vi "Config Motors NEO.vi"(8 "Reset PIDs":bool, 10 "Operation":T5, 11 "Motors In":T2 {"Steer Scaling" format="%.2f"; "Drive Scaling" format="%.2f"; "Pod Locations (ft)"."Right Back Position" format="%.2f"; "Pod Locations (ft)"."Right Front Position" format="%.2f"; "Pod Locations (ft)"."Left Back Position" format="%.2f"; "Pod Locations (ft)"."Left Front Position" format="%.2f"}) -> (3 "Motors Out":T2 {"Steer Scaling" format="%.2f"; "Drive Scaling" format="%.2f"; "Pod Locations (ft)"."Right Back Position" format="%.2f"; "Pod Locations (ft)"."Right Front Position" format="%.2f"; "Pod Locations (ft)"."Left Back Position" format="%.2f"; "Pod Locations (ft)"."Left Front Position" format="%.2f"})   [LabVIEW 2027]
uses:
  Type Definitions/Hardware/Swerve Drives/(NEO-NEO-ThroughBore-Pigeon2) Swerve.ctl
  <vilib>/REV Custom Controls/REVSparkRefnum.ctl
  Type Definitions/Data/Pod Positions.ctl
  Drive/Implementation/Drive Operations.ctl
  <vilib>/REV Custom Controls/Spark Voltage Compensation.ctl
  38a9160b-f87a-407c-aa95-d3b96145cb37.vi
  c612d860-360b-4606-b7b1-9c6eba82ec37.vi
  <resource>/objmgr/REVSpark.rc
  <vilib>/REVLibDriver/REVLibDriver.lvlib
panel:
  in  "value":bool
  in  "Immediate PID":T1={{"P Gain"=0.0005, "I Gain"=0.0, "D Gain"=0.0, "kV"=0.00175}, "I Zone"=0.0, "Output LImits"={"Min Output"=-1.0, "Max Output"=1.0}}
  in  "Auto Gains":T1={{"P Gain"=0.16, "I Gain"=0.0, "D Gain"=0.0, "kV"=0.78}, "I Zone"=0.0, "Output LImits"={"Min Output"=-1.0, "Max Output"=1.0}}
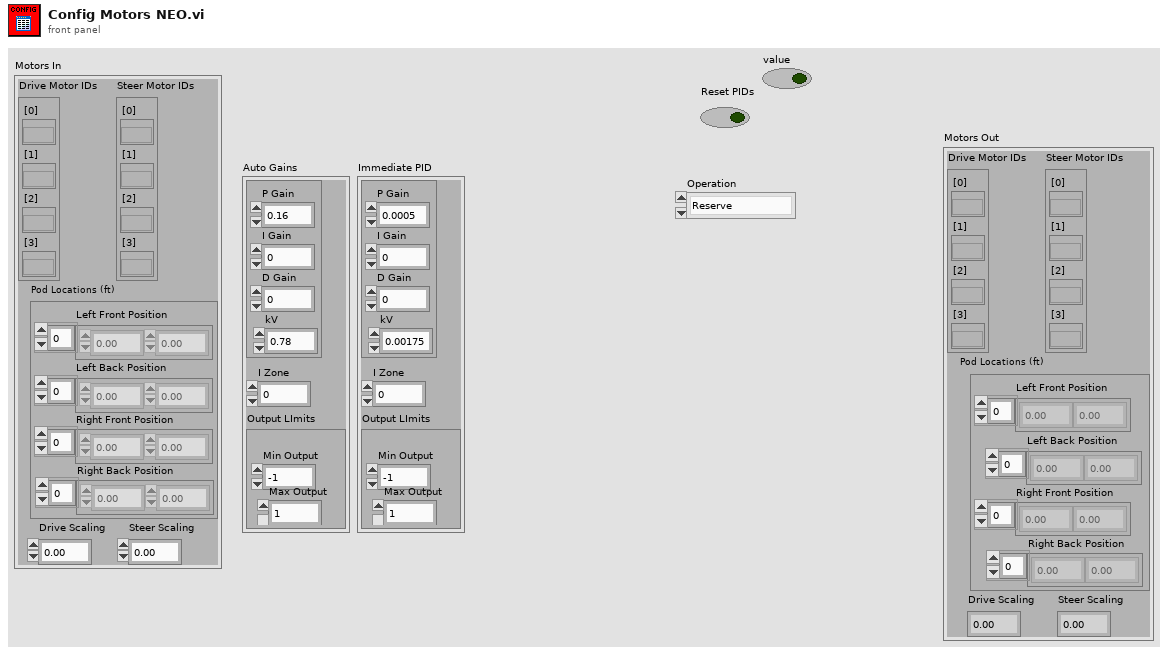
[diagram p1: front panel]
types:
  T1 = cluster{cluster{"P Gain":dbl, "I Gain":dbl, "D Gain":dbl, "kV":dbl}, "I Zone":dbl, "Output LImits":cluster{"Min Output":dbl, "Max Output":dbl}}
  T2 = typedef "(NEO-NEO-ThroughBore-Pigeon2) Swerve.ctl" = cluster{"Drive Motor IDs":cluster{"[0]":T3, "[1]":T3, "[2]":T3, "[3]":T3}, "Steer Motor IDs":cluster{"[0]":T3, "[1]":T3, "[2]":T3, "[3]":T3}, "Pod Locations (ft)":T4, "Drive Scaling":dbl, "Steer Scaling":dbl}
  T3 = typedef "REVLibDriver.lvlib/REVSparkRefnum.ctl" = refnum<k20>
  T4 = typedef "Pod Positions.ctl" = cluster{"Left Front Position":dbl[], "Left Back Position":dbl[], "Right Front Position":dbl[], "Right Back Position":dbl[]}
  T5 = typedef "Drive Operations.ctl" = enum16{"Reserve", "Read Current", "Immediate", "Calibrate", "Auto", "Auto Pickup"}
  T6 = typedef "REVLibDriver.lvlib/Spark Voltage Compensation.ctl" = cluster{"Mode":u32, "Nominal Voltage":dbl}
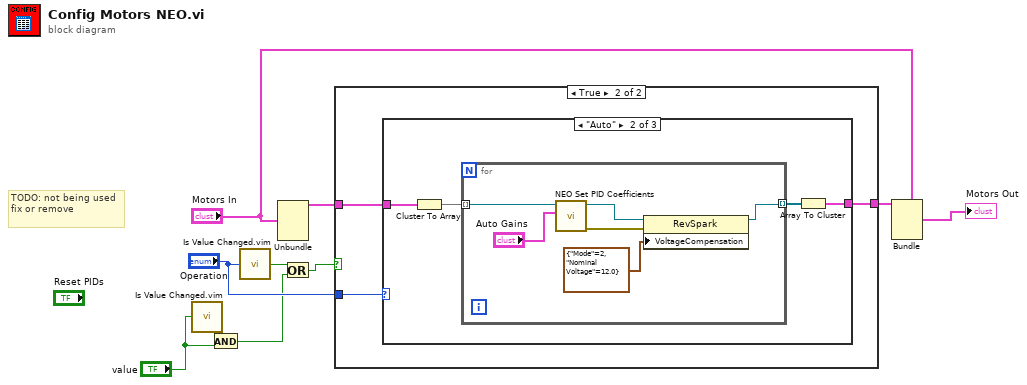
[diagram p0: block diagram]
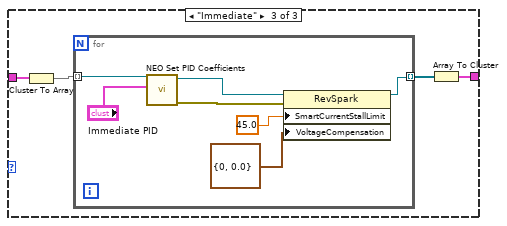
[diagram p4: hidden frame]
diagram:
  # "TODO: not being used\nfix or remove"
  n1 = call "Is Value Changed.vim"("value"="value") -> ("changed or first call?"=w3:bool)
  n2 = And(x=w3, y="value") -> (x .and. y?=w2:bool)
  n3 = call "Is Value Changed.vim"("value"="Operation") -> ("changed or first call?"=w5:bool)
  n4 = Unbundle("Motors In") -> ("Drive Motor IDs"=w10:cluster{"[0]":T3, "[1]":T3, "[2]":T3, "[3]":T3})  [unwired: 4 out]
  n5 = Or(x=w5, y=w2) -> (x .or. y?=w4:bool)
  n6 = case shown="True" w4 {
    tunnel: "Operation" -> [_ w14]
    tunnel: w10 -> [w11 w13]
    tunnel: [w11 w12] -> w8
    frame False {
    }
    frame True {
      n7 = case shown="\"Auto\"" w14 {
        tunnel: w13 -> [w15 w17 w27]
        tunnel: [w15 w18 w28] -> w12
        frame "Reserve", Default {
        }
        frame "Auto" {
          n8 = Cluster To Array(cluster=w17) -> (array=w16:T3[])
          n9 = for {
            tunnel: [w21] -> w19 mode=indexing
            tunnel: w16 -> [w25] mode=indexing
            n10 = call "NEO Set PID Coefficients.vi"("PID Gains"="Auto Gains", "Spark refnum"=w25) -> ("error out"=w20:errorcluster, "Spark refnum out"=w23:T3)  [unwired: 6 in]
            n11 = property class="RevSpark"(reference=w23, error in=w20, "VoltageCompensation"=T6 {"Mode"=2, "Nominal Voltage"=12.0}) -> (reference out=w21:T3)  [unwired: 1 out]
          }
          n12 = Array To Cluster(array=w19) -> (cluster=w18:cluster{"[0]":T3, "[1]":T3, "[2]":T3, "[3]":T3})
        }
        frame "Immediate" {
          n13 = Cluster To Array(cluster=w27) -> (array=w26:T3[])
          n14 = for {
            tunnel: w26 -> [w36] mode=indexing
            tunnel: [w31] -> w29 mode=indexing
            n15 = call "NEO Set PID Coefficients.vi"("PID Gains"="Immediate PID", "Spark refnum"=w36) -> ("error out"=w30:errorcluster, "Spark refnum out"=w32:T3)  [unwired: 6 in]
            n16 = property class="RevSpark"(reference=w32, error in=w30, "SmartCurrentStallLimit"=45.0 ("Primay Current Limit (80A)"), "VoltageCompensation"=T6 {"Mode"=0, "Nominal Voltage"=0.0}) -> (reference out=w31:T3)  [unwired: 1 out]
          }
          n17 = Array To Cluster(array=w29) -> (cluster=w28:cluster{"[0]":T3, "[1]":T3, "[2]":T3, "[3]":T3})
        }
      }
    }
  }
  n18 = Bundle(cluster="Motors In", "Drive Motor IDs"=w8) -> (→"Motors Out":T2)  [unwired: 4 in]
